vi "run.json_to_object.vi"(8 "error in":errorcluster, 11 "JSON":string) -> (0 "error out":errorcluster, 2 "Run":refnum<class "Run.lvclass">)   [LabVIEW 2020]
uses:
  Run/Run.lvclass
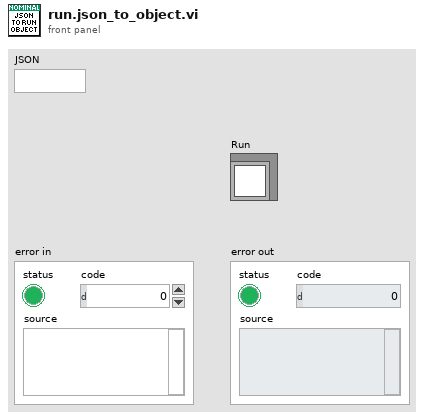
[diagram p1: front panel]
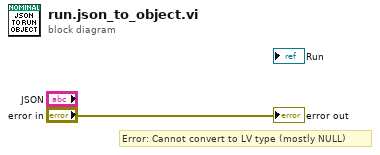
[diagram p0: block diagram]
diagram:
  # "Error: Cannot convert to LV type (mostly NULL)"
  "error out" <- "error in"
